vi "Module Loop.vi"(8 "error in (no error)":errorcluster, 11 "Remote Messaging Module in":refnum<class "Remote Messaging Module.lvclass">) -> (0 "error out":errorcluster, 3 "Remote Messaging Module out":refnum<class "Remote Messaging Module.lvclass">)   [LabVIEW 2020, in "Volatus.lvlib" / "Remote Messaging Module.lvclass"]
uses:
  Remote Messaging Module.lvclass
  C:/dev/lv20CE/relink/lv-volatus/Volatus/Module/Module.lvclass
  Module/Module.lvclass
  lv-vecto/Vecto/proto/TcpPayload/Data.ctl
  Message Forward (ID).ctl
  Module/Module.lvclass/Module.ctl
  VolatusAPI/VolatusAPI.lvclass/VolatusAPI.ctl
  Messages Registration.ctl
  MessageQ/MessageQ.lvclass
  Message Registration.ctl
  Message Unregistration.ctl
  <vilib>/Utility/error.llb/Error Cluster From Error Code.vi
  Remote Messaging Module.lvclass/Remote Messaging Module.ctl
  lv-vecto/Vecto/proto/TcpPayload/TcpPayload.lvlib
  Volatus.lvlib
  VolatusAPI/VolatusAPI.lvclass
  lv-vecto/Vecto/TCPMessageService/TCPMessageAPI.lvclass
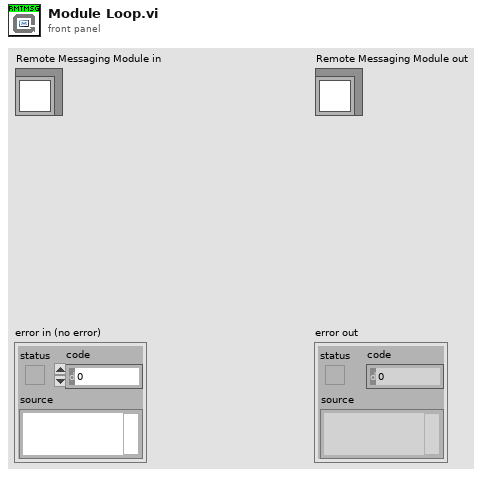
[diagram p1: front panel]
types:
  T1 = enum32{"Invalid", "Standard", "Closed", "Hidden", "Minimized", "Maximized"}
  T2 = typedef "TcpPayload.lvlib/Data.ctl" = cluster{"target_node":u32, "source_id":u32, "sequence":u32, "timestamp":i64, "type":string, "task_id":string, "payload":u8[]}
  T3 = typedef "Volatus.lvlib/Message Forward (ID).ctl" = cluster{"Node ID":u32, "Type":string, "Payload":u8[]}
  T4 = typedef "Volatus.lvlib/Messages Registration.ctl" = cluster{"MessageQ":refnum<class "MessageQ.lvclass">, "Messages":T5[]}
  T5 = typedef "Volatus.lvlib/Message Registration.ctl" = cluster{"Message Type":string, "Message ID":string}
  T6 = typedef "Volatus.lvlib/Message Unregistration.ctl" = cluster{"MessageQ":refnum<class "MessageQ.lvclass">}
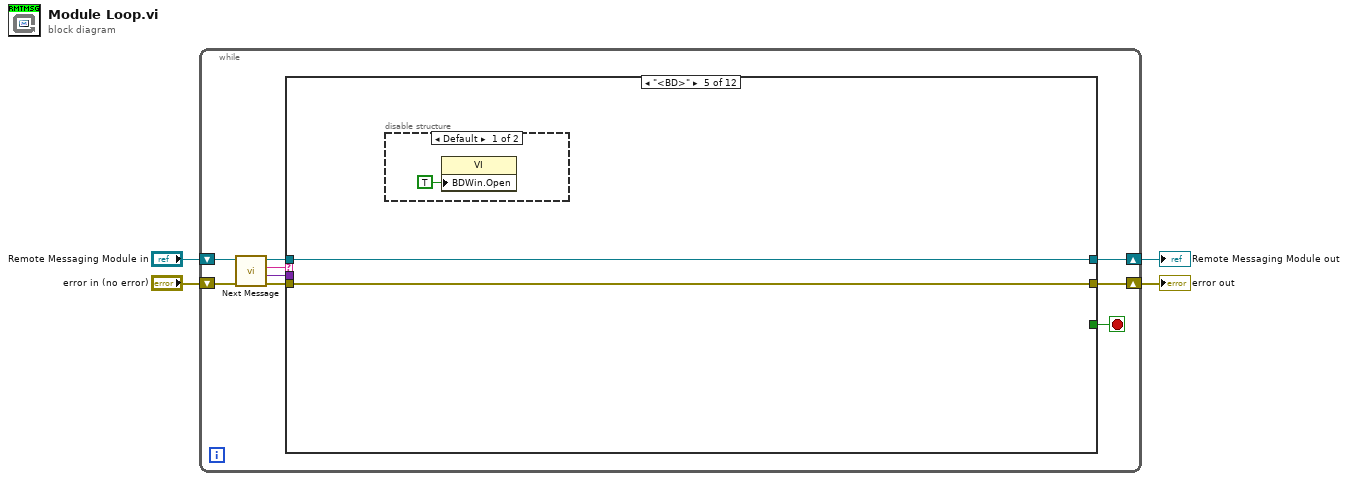
[diagram p0: block diagram]
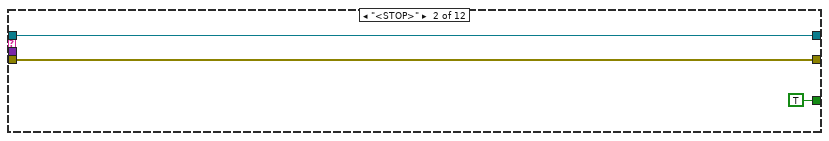
[diagram p3: hidden frame]
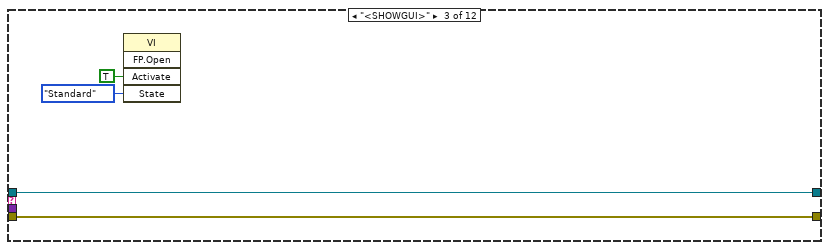
[diagram p4: hidden frame]
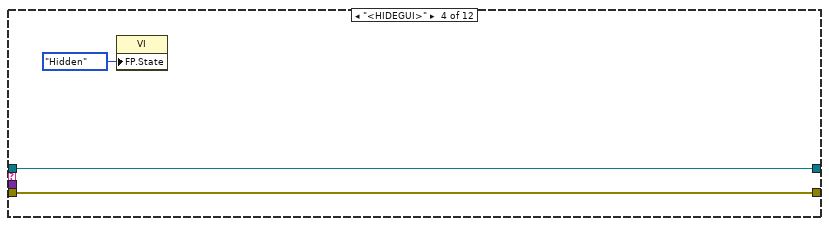
[diagram p5: hidden frame]
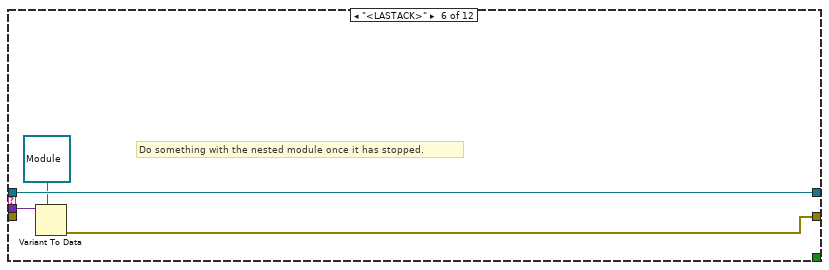
[diagram p7: hidden frame]
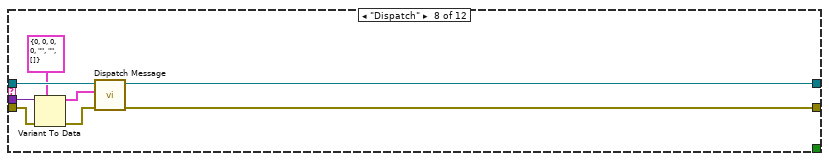
[diagram p9: hidden frame]
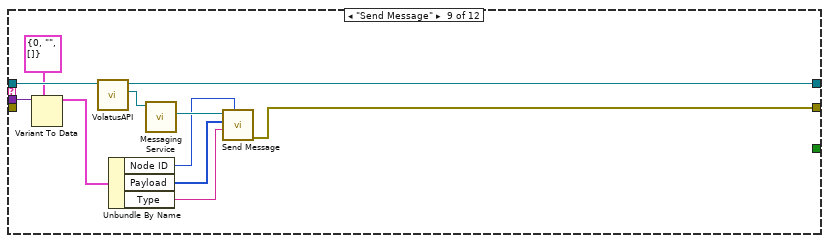
[diagram p10: hidden frame]
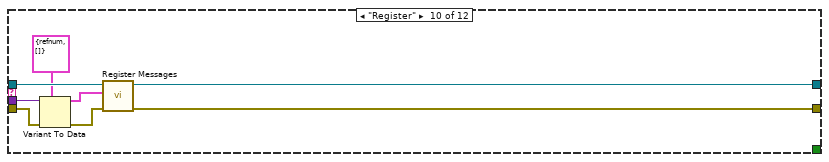
[diagram p11: hidden frame]
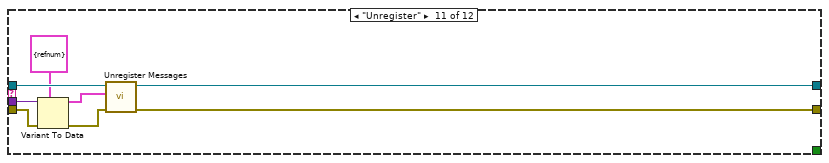
[diagram p12: hidden frame]
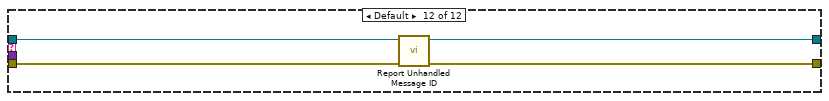
[diagram p13: hidden frame]
diagram:
  n1 = while {
    shift-right: [w8] -> w1
    shift-left: "Remote Messaging Module in" -> [w13]
    shift-right: [w7] -> w2
    shift-left: "error in (no error)" -> [w12]
    stop <- w6 stop-if-true
    n2 = call "Next Message.vi"("error in (no error)"=w12, "Module in"=w13) -> ("error out"=w11:errorcluster, "Data"=w5:variant, "ID"=w10:string, "Module out"=w9:refnum<class "Remote Messaging Module.lvclass">)  [unwired: 6 in]
    n3 = case shown="\"<BD>\"" w10 {
      tunnel: w11 -> [w14 w17 w21 w24 w26 _ w33 w40 _ w59 w68 w73]
      tunnel: w9 -> [w15 w18 w22 w25 w27 w32 w34 w42 w53 w61 w69 w71]
      tunnel: [w15 w18 w22 w25 w27 w32 w34 w38 w49 w57 w65 w70] -> w8
      tunnel: [w14 w17 w21 w24 w26 w29 w33 w35 w43 w54 w63 w72] -> w7
      tunnel: [_ TRUE _ _ _ _ _ _ _ _ _ _] -> w6
      tunnel: w5 -> [_ _ _ _ _ w31 _ w41 w52 w60 w67 _]
      frame "<CLOSE>" {
      }
      frame "<STOP>" {
      }
      frame "<SHOWGUI>" {
        n4 = invoke class="VI" method="FP.Open"("Activate"=TRUE ("Activate?"), "State"=T1."Standard") -> ()  [unwired: 3 in, 5 out]
      }
      frame "<HIDEGUI>" {
        n5 = property class="VI"("FP.State"=T1."Hidden" ("Front Panel Window:State")) -> ()  [unwired: 2 in, 2 out]
      }
      frame "<BD>" {
        n6 = disable-structure shown="Default" {
          frame condition #0 (active) {
            n7 = property class="VI"("BDWin.Open"=TRUE ("Block Diagram Window:Open")) -> ()  [unwired: 2 in, 2 out]
          }
          frame condition #1 {
          }
        }
      }
      frame "<LASTACK>" {
        # "Do something with the nested module once it has stopped."
        n8 = Variant To Data(type=refnum<class "Module.lvclass"> refnum ("Volatus:Module"), Variant=w31) -> (error out=w29:errorcluster)  [unwired: 1 in, 1 out]
      }
      frame "<TIMEOUT>" {
        # "No message for this module was received in time"
      }
      frame "Dispatch" {
        n9 = Variant To Data(error in=w40, type=T2 {"target_node"=0, "source_id"=0, "sequence"=0, "timestamp"=0, "type"="", "task_id"="", "payload"=[]} ("TcpPayload"), Variant=w41) -> (data=w37:T2, error out=w36:errorcluster)
        n10 = call "Dispatch Message.vi"("error in (no error)"=w36, "TcpPayload"=w37, "Remote Messaging Module in"=w42) -> ("error out"=w35:errorcluster, "Remote Messaging Module out"=w38:refnum<class "Remote Messaging Module.lvclass">)  [unwired: 7 in]
      }
      frame "Send Message" {
        n11 = Variant To Data(type=T3 {"Node ID"=0, "Type"="", "Payload"=[]} ("Message Forward (ID)"), Variant=w52) -> (data=w50:T3)  [unwired: 1 in, 1 out]
        n12 = call "VolatusAPI.vi"("Module in"=w53) -> ("VolatusAPI"=w48:refnum<class "VolatusAPI.lvclass">, "Module out"=w49:refnum<class "Remote Messaging Module.lvclass">)  [unwired: 9 in]
        n13 = Unbundle By Name(w50) -> ("Node ID"=w44:u32, "Payload"=w46:u8[], "Type"=w45:string)
        n14 = call "Messaging Service.vi"("VolatusAPI in"=w48) -> ("Messaging"=w47:refnum<class "TCPMessageAPI.lvclass">)  [unwired: 8 in, 2 out]
        n15 = call "Send Message.vi"("Target ID"=w44, "Type"=w45, "Payload"=w46, "TCPMessageService in"=w47) -> ("error out"=w43:errorcluster)  [unwired: 6 in, 1 out]
      }
      frame "Register" {
        n16 = Variant To Data(error in=w59, type=T4 {"MessageQ"=refnum, "Messages"=[]} ("Messages Registration"), Variant=w60) -> (data=w56:T4, error out=w55:errorcluster)
        n17 = call "Register Messages.vi"("error in (no error)"=w55, "Messages Registration"=w56, "Remote Messaging Module in"=w61) -> ("error out"=w54:errorcluster, "Remote Messaging Module out"=w57:refnum<class "Remote Messaging Module.lvclass">)  [unwired: 7 in]
      }
      frame "Unregister" {
        n18 = Variant To Data(error in=w68, type=T6 {"MessageQ"=refnum} ("Message Unregistration"), Variant=w67) -> (data=w62:T6, error out=w64:errorcluster)
        n19 = call "Unregister Messages.vi"("error in (no error)"=w64, "Message Unregistration"=w62, "Remote Messaging Module in"=w69) -> ("error out"=w63:errorcluster, "Remote Messaging Module out"=w65:refnum<class "Remote Messaging Module.lvclass">)  [unwired: 7 in]
      }
      frame Default {
        n20 = call "Report Unhandled Message ID.vi"("error in (no error)"=w73, "Module in"=w71) -> ("error out"=w72:errorcluster, "Module out"=w70:refnum<class "Remote Messaging Module.lvclass">)  [unwired: 8 in]
      }
    }
  }
  "error out" <- w2
  "Remote Messaging Module out" <- w1
